vi "Write DAQ FIFO.vi"(6 "FIFO Timestamps":T2, 8 "error in (no error)":errorcluster, 9 "Timeout (ms)":i32, 10 "Data In":T1[](array[typedef]), 11 "CIFFIFO in":refnum<class "CIF_Iceoryx_Fifo_DAQ.lvclass">) -> (0 "error out":errorcluster, 1 "timed out?":bool, 2 "Data Out":T1[](array[typedef]), 3 "CIFFIFO out":refnum<class "CIF_Iceoryx_Fifo_DAQ.lvclass">)   [LabVIEW 2021, in "CIF_Iceoryx_Fifo_DAQ.lvclass"]
uses:
  CIF_Iceoryx_Fifo_DAQ.lvclass
  ChannelCommon/typedef/TimeStamps.ctl
  D:/dev/Packages/CIF_Channels_Core/src/Iceorxy_Channels/PCAP_Universal/CIF_Iceoryx_PCAP_Universal.lvclass
  D:/dev/Packages/CIF_Channels_Core/src/CIFChannels/CIFChannels.lvclass
  ChannelCommon/typedef/Datatype Waveform.ctl
  PCAP_Universal/CIF_Iceoryx_PCAP_Universal.lvclass/CIF_Iceoryx_PCAP_Universal.ctl
  <vilib>/CIF Foundation/CIF Utilities/DataTypes/Typedef/Endian.ctl
  <vilib>/CIF Foundation/CIF PCAP Parse and Build/pcap_Parse_Build_CIF.lvclass
  <vilib>/CIF Foundation/CIF PCAP Parse and Build/pcap_Parse_Build_CIF.lvclass/pcap_Parse_Build_CIF.ctl
  <vilib>/CIF Foundation/CIF PCAP DAQ/typedef/DAQ Header.ctl
  <vilib>/CIF Foundation/CIF PCAP DAQ/typedef/Interleaved.ctl
  CIFChannels/CIFChannels.lvclass/CIFChannels.ctl
  <vilib>/CIF Foundation/CIF Utilities/Statistics/I64/Stats_I64_CIF_U.lvclass/Stats_I64_CIF_U.ctl
  0d20d4f4-e248-4459-b628-727107c05f7a.vi
  2d5faa5a-4fe5-40e6-9038-fec4d205edfd.vi
  725f190d-4de5-499c-bccf-8cc742c86a22.vi
  PCAP_Universal/Accessors/Read Payload.vi
  <vilib>/CIF Foundation/CIF PCAP Parse and Build/Data Accessors/Write OS Endian.vi
  PCAP_Universal/Accessors/Write Payload.vi
  <vilib>/CIF Foundation/CIF PCAP Parse and Build/Build/SubVIs/Flatten Packet Header.vi
  <vilib>/CIF Foundation/CIF Utilities/Statistics/I64/X1 minus X0.vi
  0d20d4f4-e248-4459-b628-727107c05f7a.vi/c28b0ead-42ad-4072-80a2-aca7f2bd7ce3.vi
  0d20d4f4-e248-4459-b628-727107c05f7a.vi/d83f0d1e-b5f2-409c-a855-55c666a7c55e.vi
  0d20d4f4-e248-4459-b628-727107c05f7a.vi/c4136907-e772-4046-b7cd-6e4b8d78dccc.vi
  <vilib>/CIF Foundation/CIF Utilities/Time/System Time/Get System Time.vi
  <vilib>/CIF Foundation/CIF Utilities/DataTypes/Flatten Unflatten/Flatten U32.vi
  <vilib>/CIF Foundation/CIF Utilities/Statistics/I64/X1 minus X0.vi/dfabcf33-0dbc-4041-80a5-3dc0c86d2989.vi
  <vilib>/CIF Foundation/CIF Utilities/Time/System Time/LabVIEW Time to TAI Time.vi
  <vilib>/CIF Foundation/CIF Utilities/Statistics/I64/X1 minus X0.vi/dfabcf33-0dbc-4041-80a5-3dc0c86d2989.vi/9eb60a9a-770f-4d2d-8b3f-8465c267ecc9.vi
  CIF_Iceoryx_Fifo_DAQ.lvclass/CIF_Iceoryx_Fifo_DAQ.ctl
  <vilib>/CIF Foundation/CIF PCAP DAQ/PCAP DAQ Core.lvlib
  <vilib>/CIF Foundation/CIF Utilities/DataTypes/DataTypes_CIF_U.lvlib
  CIFChannels/CIFChannels.lvclass
  ChannelCommon/ChannelCommon.lvlib
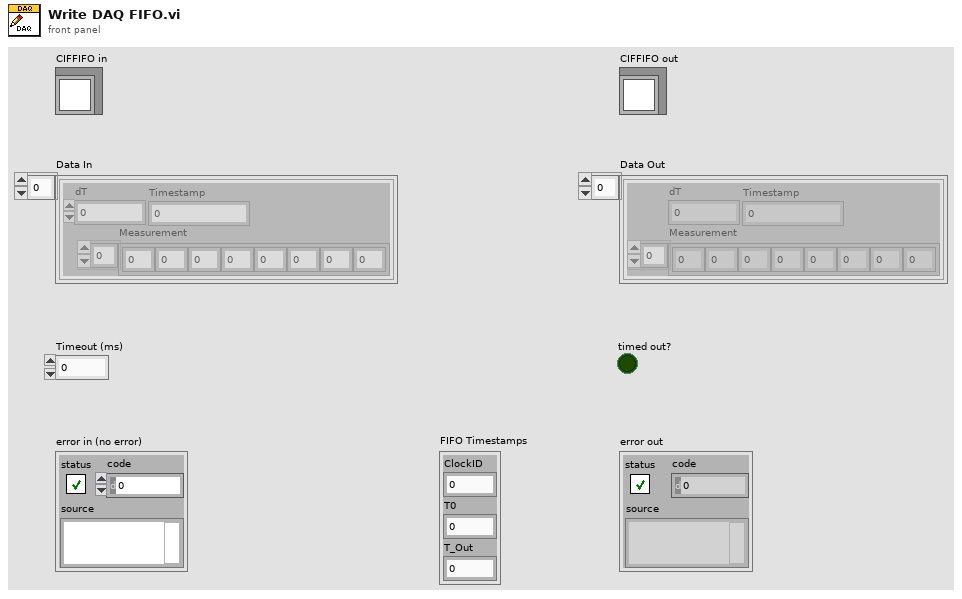
[diagram p1: front panel]
types:
  T1 = typedef "ChannelCommon.lvlib/Datatype Waveform.ctl" = cluster{"Measurement":dbl[], "dT":dbl, "Timestamp":i64}
  T2 = typedef "ChannelCommon.lvlib/TimeStamps.ctl" = cluster{"ClockID":u8, "T0":i64, "T_Out":i64}
  T3 = typedef "DataTypes_CIF_U.lvlib/Endian.ctl" = enum16{"Little Endian", "Big Endian"}
  T4 = typedef "PCAP DAQ Core.lvlib/DAQ Header.ctl" = cluster{"dT (s)":dbl, "Channels":u16, "Endian":enum16{"Little Endian", "Big Endian"}, "Interleaved":T5}
  T5 = typedef "PCAP DAQ Core.lvlib/Interleaved.ctl" = enum8{"Concatenated", "Interleaved"}
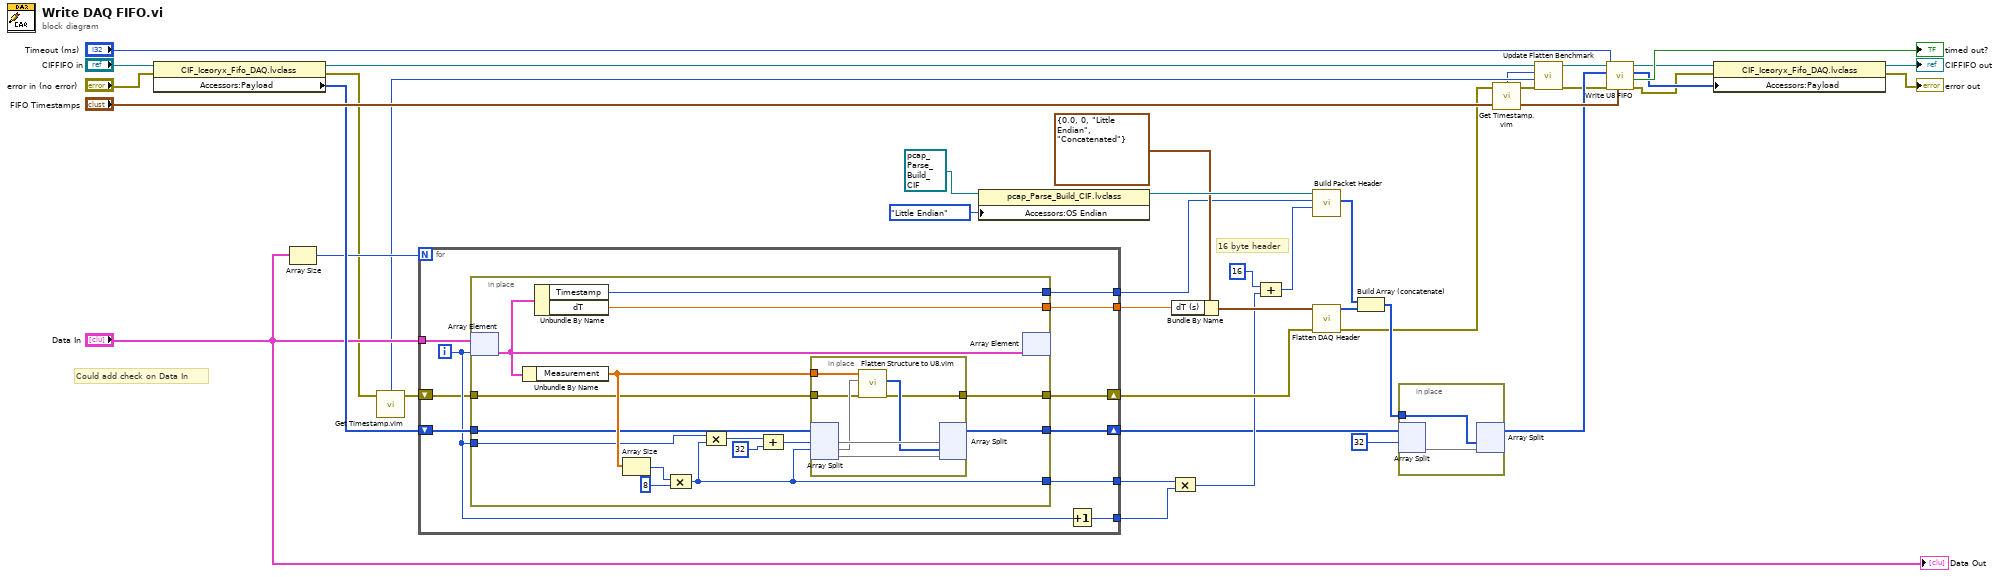
[diagram p0: block diagram]
diagram:
  # "Could add check on Data In"
  # "16 byte header"
  n1 = property class="CIF_Iceoryx_Fifo_DAQ.lvclass"(reference="CIFFIFO in", error in="error in (no error)") -> (reference out=w12:refnum<class "CIF_Iceoryx_Fifo_DAQ.lvclass">, error out=w6:errorcluster, "Accessors:Payload"=w37:u8[])
  n2 = Array Size(array="Data In") -> (size(s)=w36:i32)
  n3 = call "Get Timestamp.vim"("Anything in"=w6) -> ("Time (ns)"=w5:i64, "Anything out"=w4:errorcluster)  [unwired: 2 in]
  n4 = for {
    N: w36 -> [_]
    shift-right: [w49] -> w9
    shift-left: w37 -> [w51]
    shift-right: [w42] -> w23
    shift-left: w4 -> [w43]
    tunnel: [w48] -> w24
    tunnel: [w47] -> w25
    tunnel: [w46] -> w20
    tunnel: [w44] -> w18
    tunnel: "Data In" -> [w50]
    i -> [w45]
    n5 = in-place {
      in-place-border: w51 -> [w59]
      in-place-border: w45 -> [w61]
      in-place-border: [w58] -> w49
      in-place-border: w43 -> [w52]
      in-place-border: [w53] -> w42
      in-place-border: [w57] -> w48
      in-place-border: [w56] -> w47
      in-place-border: [w55] -> w46
      n6 = in-place-array #1(w50, w45) -> (w54:T1)
      n7 = Unbundle By Name(w54) -> ("Measurement"=w64:dbl[])
      n8 = Unbundle By Name(w54) -> ("Timestamp"=w57:i64, "dT"=w56:dbl)
      n9 = Array Size(array=w64) -> (size(s)=w66:i32)
      n10 = Compound Arithmetic op=MULTIPLY(w66, 8 ("value")) -> (w55:i32)
      n11 = Compound Arithmetic op=MULTIPLY(w61, w55) -> (w63:i32)
      n12 = Compound Arithmetic op=ADD(w63, 32 ("value")) -> (w60:i32)
      n13 = in-place {
        in-place-border: w52 -> [w67]
        in-place-border: w64 -> [w73]
        in-place-border: [w68] -> w53
        n14 = in-place-split #2(w59, w60, w55) -> (w72:u8[], w70:u8[], w71:u8[])
        n15 = call "Flatten Structure to U8.vim"("error in"=w67, "Flattened Data in"=w70, "Data to Flatten in"=w73) -> ("error out"=w68:errorcluster, "Flattened Data out"=w69:u8[])  [unwired: 6 in, 1 out]
        n16 = in-place-split #2(w72, w69, w71) -> (w58:u8[])  [unwired: 2 out]
      }
      n17 = in-place-array #1(w54) -> ()  [unwired: 2 out]
    }
    n18 = Increment(x=w45) -> (x+1=w44:i32)
  }
  n19 = property class="pcap_Parse_Build_CIF.lvclass"(reference=refnum<class "pcap_Parse_Build_CIF.lvclass"> refnum ("pcap Parse and Build in"), "Accessors:OS Endian"=Endian."Little Endian" ("OS Endian")) -> (reference out=w34:refnum<class "pcap_Parse_Build_CIF.lvclass">)  [unwired: 1 in, 1 out]
  n20 = Bundle By Name(cluster=T4 {"dT (s)"=0.0, "Channels"=0, "Endian"=enum."Little Endian", "Interleaved"=enum."Concatenated"} ("DAQ Header"), "dT (s)"=w25) -> (w29:T4)
  n21 = Compound Arithmetic op=MULTIPLY(w20, w18) -> (w19:i32)
  n22 = Compound Arithmetic op=ADD(16 ("x"), w19) -> (w27:i32)
  n23 = call <vilib>:"Build Packet Header.vi"("Length"=w27, "TAI Time (ns)"=w24, "pcap Parse and Build in"=w34) -> ("Flattened Data out"=w30:u8[])  [unwired: 7 in, 1 out]
  n24 = call <vilib>:"Flatten DAQ Header.vi"("error in"=w23, "DAQ Header"=w29) -> ("error out"=w2:errorcluster, "Flat DAQ Header"=w31:u8[])  [unwired: 8 in]
  n25 = Build Array (concatenate)(w30, w31) -> (w8:u8[])
  n26 = in-place {
    in-place-border: w8 -> [w74]
    n27 = in-place-split #3(w9, 32) -> (w75:u8[])  [unwired: 1 out]
    n28 = in-place-split #3(w74, w75) -> (w22:u8[])  [unwired: 1 out]
  }
  n29 = call "Get Timestamp.vim"("Anything in"=w2) -> ("Time (ns)"=w3:i64, "Anything out"=w1:errorcluster)  [unwired: 2 in]
  n30 = call "Update Flatten Benchmark.vi"("error in (no error)"=w1, "X0"=w5, "X1"=w3, "CIFChannels in"=w12) -> ("error out"=w10:errorcluster, "CIFChannels out"=w11:refnum<class "CIF_Iceoryx_Fifo_DAQ.lvclass">)  [unwired: 6 in]
  n31 = call-dynamic "Write U8 FIFO.vi"("FIFO Timestamps"="FIFO Timestamps", "error in (no error)"=w10, "Timeout (ms)"="Timeout (ms)", "Data in"=w22, "CIFFIFO in"=w11) -> ("error out"=w13:errorcluster, "timed out?"=→"timed out?":bool, "Data out"=w16:u8[], "CIFFIFO out"=w17:refnum<class "CIF_Iceoryx_Fifo_DAQ.lvclass">)  [unwired: 3 in]
  n32 = property class="CIF_Iceoryx_Fifo_DAQ.lvclass"(reference=w17, error in=w13, "Accessors:Payload"=w16) -> (reference out=→"CIFFIFO out":refnum<class "CIF_Iceoryx_Fifo_DAQ.lvclass">, error out=→"error out":errorcluster)
  "Data Out" <- "Data In"
